vi "PicoScope4000aExampleRapidBlockBulkOverlapped.vi"() -> ()   [LabVIEW 2010]
doc: "This example demonstrates how to use the PicoScope Labview library to collect data using rapid block mode, retrieving the data values in bulk."
uses:
  shared/PicoBuffers.ctl
  PicoScope4000aLib/PicoScope4000aAnalogChannelSettings.ctl
  shared/Segment Range.ctl
  shared/Buffer and Transfer Settings.ctl
  shared/Acquisition Settings.ctl
  shared/nSegments.ctl
panel:
  in  "Resolution":u32(ring)=1 items=["8-bit", "12-bit", "14-bit"]
  out "Unit Info":T1
  in  "Trigger Settings":T2={"Trigger Enabled"=FALSE, "Trigger Source"=enum."Channel A", "Trigger Threshold (Volts/Probe units)"=0.0, "Trigger Direction"=2, "Trigger Delay (samples)"=0, "Auto Trigger Time (ms)"=1000} {"Trigger Direction" items=["Rising"=2, "Falling"=3]}
  out "overflow":i16[](array[numeric]) format="%08b"
  in  "Channel A Settings":T3={"Enabled"=TRUE, "Coupling"=1, "Range"=6, "Analogue Offset"=0.0, "Bandwidth Limit"=0} {"Bandwidth Limit" items=["Full", "20kHz", "100kHz", "1MHz"]; "Range" items=["10 mV", "20 mV", "50 mV", "100 mV", "200 mV", "500 mV", "1 V", "2 V", "5 V", "10 V", "20 V", "50 V ", "100 V"]; "Coupling" items=["AC", "DC"]}
  out "USB 3.0 device on non-USB 3.0 Port":bool
  out "USB Powered":bool=TRUE
  in  "Stop Display":bool
  out "Capture Complete":bool
  in  "Run":bool
  in  "Display Buffer Index":i32
  in  "Segment Range":T4={"fromSegmentIndex"=0, "toSegmentIndex"=9} {"toSegmentIndex" format="%.4p"; "fromSegmentIndex" format="%.4p"}
  in  "nSegments":T5=10 format="%.4p"
  out "error out":errorcluster
  in  "Data file":path=path "PicoScope4000aExampleRapidBlock ChA Data"
  in  "Buffer and Transfer Settings":T6={"startIndex"=0, "Samples"=5000000, "Down Sample Ratio"=1, "Down-Sample Mode"=0} {"Down-Sample Mode" items=["RAW none"=2147483648, "None"=0, "Aggregate"=1, "Decimate"=2, "Average"=4]; "Down Sample Ratio" step=1; "Samples" format="%_6p"}
  in  "Acquisition Settings":T7={"preTriggerSamples"=0, "postTriggerSamples"=5000000, "timebase"=5} {"postTriggerSamples" format="%_6p"; "preTriggerSamples" format="%_6p"}
  out "Properties Panel":T8={"Sample Frequency"=41666668.0, "Sample Rate"=2.4000000209412065e-08, "Max Samples Available"=26843008, "Number of Samples"=0, "Total Capture Time (sec) "=0.0, "Max Total Capture Time Available (sec)"=0.6442322134971619} {"Max Total Capture Time Available (sec)" format="%.3p"; "Sample Frequency" format="%.6p"; "Sample Rate" format="%.3p"; "Max Samples Available" format="%_6p"; "Total Capture Time (sec)" format="%.3p"}
  in  "stop":bool
  out "Analog Channels":cluster{i32, dbl, "Data":dbl[]}[](graph)
  in  "Serial Number":string
  in  "Use Serial Number":bool
  in  "error in (no error)":errorcluster
  # "Number of\nSegments to Capture"
  # "Bit 0 = ChA"
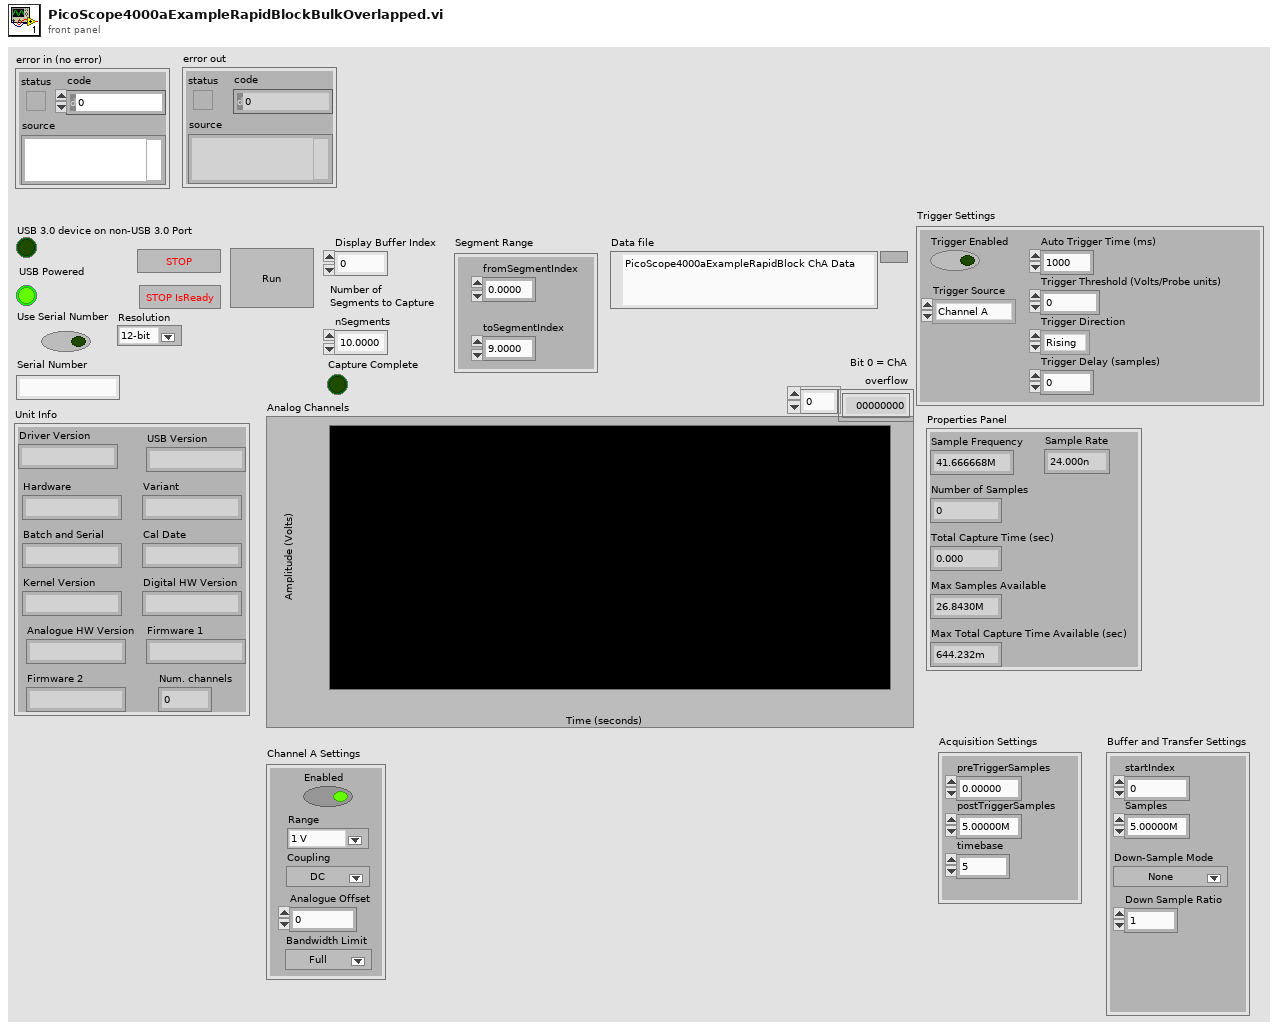
[diagram p1: front panel]
types:
  T1 = cluster{"Driver Version":string, "USB Version":string, "Hardware":string, "Variant":string, "Batch and Serial":string, "Cal Date":string, "Kernel Version":string, "Digital HW Version":string, "Analogue HW Version":string, "Firmware 1":string, "Firmware 2":string, "Num. channels":i16}
  T2 = cluster{"Trigger Enabled":bool, "Trigger Source":enum16{"Channel A", "Channel B", "Channel C", "Channel D", "Channel E", "Channel F", "Channel G", "Channel H"}, "Trigger Threshold (Volts/Probe units)":dbl, "Trigger Direction":u16, "Trigger Delay (samples)":u32, "Auto Trigger Time (ms)":i16}
  T3 = typedef "PicoScope4000aAnalogChannelSettings.ctl" = cluster{"Enabled":bool, "Coupling":i16, "Range":u16, "Analogue Offset":sgl, "Bandwidth Limit":u32}
  T4 = typedef "Segment Range.ctl" = cluster{"fromSegmentIndex":u64, "toSegmentIndex":u64}
  T5 = typedef "nSegments.ctl" = u64
  T6 = typedef "Buffer and Transfer Settings.ctl" = cluster{"startIndex":u64, "Samples":u64, "Down Sample Ratio":u64, "Down-Sample Mode":u32}
  T7 = typedef "Acquisition Settings.ctl" = cluster{"preTriggerSamples":u64, "postTriggerSamples":u64, "timebase":u32}
  T8 = cluster{"Sample Frequency":dbl, "Sample Rate":dbl, "Max Samples Available":u64, "Number of Samples":u64, "Total Capture Time (sec) ":dbl, "Max Total Capture Time Available (sec)":dbl}
  T9 = enum16{"open", "open or create", "create or replace", "create", "open (read-only)"}
  T10 = typedef "PicoBuffers.ctl" = cluster{"Max Buffer Pointers":u64[][][], "Min Buffer Pointers":u64[][][], "StreamingDataInfo":cluster{"Channel":u32, "Down-Sample Mode":u32, "PICO_DATA_TYPE":enum32{"PICO_INT8_T", "PICO_INT16_T", "PICO_INT32_T", "PICO_UINT32_T", "PICO_INT64_T", ""}, "Samples":i32, "bufferIndex":u64, "startIndex":i32, "overflow":i16}[][]}
  T11 = cluster{"Channel A Buffer":i16[], "Channel B Buffer":i16[], "Channel C Buffer":i16[], "Channel D Buffer":i16[], "Channel E Buffer":i16[], "Channel F Buffer":i16[], "Channel G Buffer":i16[], "Channel H Buffer":i16[], "Port 0 Buffer":i16[], "Port 1 Buffer":i16[]}[]
  T12 = cluster{"Channel A Buffer":i16[], "Channel B Buffer":i16[], "Channel C Buffer":i16[], "Channel D Buffer":i16[], "Channel E Buffer":i16[], "Channel F Buffer":i16[], "Channel G Buffer":i16[], "Channel H Buffer":i16[], "Port 0 Buffer":i16[], "Port 1 Buffer":i16[]}
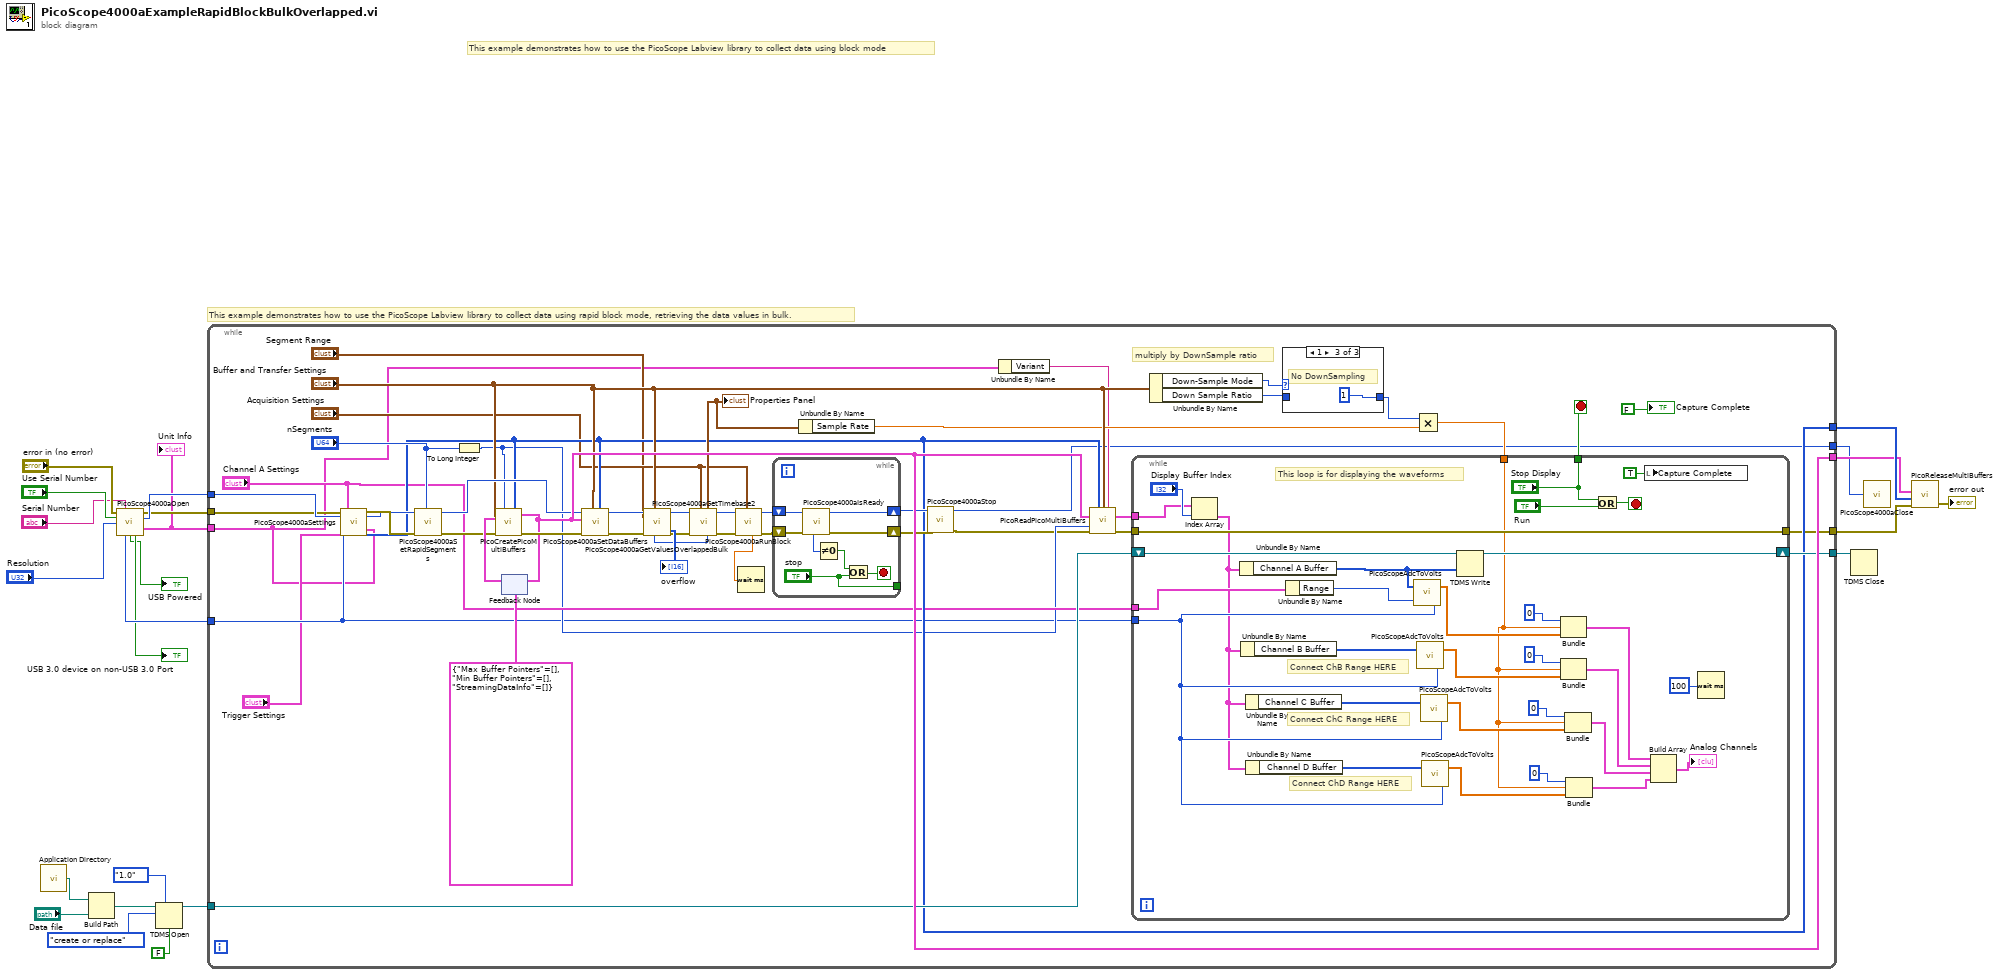
[diagram p0: block diagram]
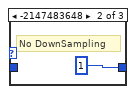
[diagram p3: hidden frame]
diagram:
  # "This example demonstrates how to use the PicoScope Labview library to collect data using rapid block mode, retrieving the data values in bulk."
  # "This example demonstrates how to use the PicoScope Labview library to collect data using block mode"
  n1 = call <vilib>:"Application Directory.vi"() -> ("Application Directory"=w14:path)
  n2 = Build Path(base path=w14, name or relative path="Data file") -> (appended path=w15:path)
  n3 = call "PicoScope4000aOpen.vi"("error in (no error)"="error in (no error)", "Serial Number"="Serial Number", "Use Serial Number"="Use Serial Number", "Resolution"="Resolution") -> ("error out"=w8:errorcluster, "handle"=w23:i16, "Unit Info"=w6:T1, "Max ADC value"=w9:i16, "USB powered"=→"USB Powered":bool, "USB 3.0 on non-USB 3.0 port"=→"USB 3.0 device on non-USB 3.0 Port":bool)  [unwired: 6 in]
  "Unit Info" <- w6
  n4 = TDMS Open(6:FALSE ("disable buffering? (T)"), 7:enum16{"1.0", "2.0"}."1.0" ("file format version (2.0)"), 10:T9."create or replace" ("operation (0:open)"), 11:w15) -> (3:w12:refnum<k34>)  [unwired: 2 in, 1 out]
  n5 = while {
    tunnel: w23 -> [w45]
    tunnel: w9 -> [w37]
    tunnel: [w26] -> w20
    tunnel: [w43] -> w22
    tunnel: [w69] -> w21
    tunnel: [w68] -> w13
    tunnel: w12 -> [w67]
    tunnel: w6 -> [w32]
    tunnel: w8 -> [w44]
    tunnel: [w42] -> w7
    stop <- w52 stop-if-true
    # "multiply by DownSample ratio"
    n6 = call "PicoScope4000aSettings.vi"("error in"=w44, "handle in"=w45, "Max ADC value"=w37, "Trigger Settings"="Trigger Settings", "Channel A Settings"="Channel A Settings", "Unit Info"=w32) -> ("error out"=w47:errorcluster, "handle out"=w46:i16, "Enabled array"=w43:i16[])  [unwired: 11 in]
    n7 = call "PicoScope4000aSetRapidSegments.vi"("nSegments"="nSegments", "error in (no error)"=w47, "handle in"=w46) -> ("error out"=w66:errorcluster, "handle out"=w65:i16)  [unwired: 6 in, 1 out]
    n8 = To Long Integer(number="nSegments") -> (32bit integer=w40:i32)
    n9 = feedback #1(T10 {"Max Buffer Pointers"=[], "Min Buffer Pointers"=[], "StreamingDataInfo"=[]} ("Data Pointers")) -> (w71:T10)
    n10 = call "PicoCreatePicoMultiBuffers.vi"("Number of Buffers"=w40, "Buffer and Transfer Settings"="Buffer and Transfer Settings", "enabled array"=w43, "Data Pointers In"=w71, "error in (no error)"=w66) -> ("Data Pointers"=w69:T10, "error out"=w70:errorcluster)  [unwired: 9 in]
    n11 = feedback-in #1(w69) -> ()
    n12 = call "PicoScope4000aSetDataBuffers.vi"("enabled array"=w43, "Buffer and Transfer Settings"="Buffer and Transfer Settings", "error in (no error)"=w70, "Data Pointers In"=w69, "handle in"=w65) -> ("error out"=w64:errorcluster, "handle out"=w63:i16)  [unwired: 5 in]
    n13 = call "PicoScope4000aGetValuesOverlappedBulk.vi"("Segment Range"="Segment Range", "Buffer and Transfer Settings"="Buffer and Transfer Settings", "error in (no error)"=w64, "handle in"=w63) -> ("error out"=w30:errorcluster, "handle out"=w31:i16, "overflow"=→"overflow":i16[], "noOfSamples"=w25:u64)  [unwired: 4 in]
    n14 = call "PicoScope4000aGetTimebase2.vi"("Number of Samples"=w25, "Acquisition Settings"="Acquisition Settings", "error in (no error)"=w30, "handle in"=w31) -> ("error out"=w28:errorcluster, "handle out"=w29:i16, "Properties Panel"=w58:T8)  [unwired: 5 in]
    "Properties Panel" <- w58
    n15 = call "PicoScope4000aRunBlock.vi"("Acquisition Settings"="Acquisition Settings", "error in (no error)"=w28, "handle in"=w29) -> ("error out"=w55:errorcluster, "handle out"=w54:i16, "timeIndisposedMs"=w24:dbl)  [unwired: 5 in, 1 out]
    n16 = Wait (ms)(milliseconds to wait=w24) -> ()  [unwired: 1 out]
    n17 = while {
      shift-right: [w111] -> w49
      shift-left: w55 -> [w112]
      shift-right: [w110] -> w48
      shift-left: w54 -> [w109]
      tunnel: ["stop"] -> _
      stop <- w106 stop-if-true
      n18 = call "PicoScope4000aIsReady.vi"("error in (no error)"=w112, "handle in"=w109) -> ("error out"=w111:errorcluster, "handle out"=w110:i16, "ready"=w108:i16)  [unwired: 7 in]
      n19 = Not Equal To 0?(x=w108) -> (x != 0?=w107:bool)
      n20 = Or(x=w107, y="stop") -> (x .or. y?=w106:bool)
    }
    n21 = Unbundle By Name(w58) -> ("Sample Rate"=w35:dbl)
    n22 = call "PicoScope4000aStop.vi"("error in (no error)"=w49, "handle in"=w48) -> ("error out"=w27:errorcluster, "handle out"=w26:i16)  [unwired: 8 in]
    n23 = Unbundle By Name(w32) -> ("Variant"=w34:string)
    n24 = call "PicoReadPicoMultiBuffers.vi"("enabled array"=w43, "Buffer and Transfer Settings"="Buffer and Transfer Settings", "Variant"=w34, "Data Pointers"=w69, "No of Buffers"=w40, "error in (no error)"=w27) -> ("MultiBuffers (Max or non-aggregated)"=w61:T11, "error out"=w53:errorcluster)  [unwired: 7 in, 1 out]
    n25 = Unbundle By Name("Buffer and Transfer Settings") -> ("Down-Sample Mode"=w59:u32, "Down Sample Ratio"=w60:u64)
    n26 = case shown="1" w59 {
      tunnel: [w113 u64 1 ("Down Sample Ratio") u64 1 ("Down Sample Ratio")] -> w56
      tunnel: w60 -> [w113 _ _]
      frame Default {
      }
      frame -2147483648 {
        # "No DownSampling"
      }
      frame 1 {
        # "No DownSampling"
      }
    }
    n27 = Multiply(x=w56, y=w35) -> (x*y=w57:dbl)
    n28 = while {
      tunnel: w37 -> [w74]
      tunnel: "Channel A Settings" -> [w104]
      tunnel: w61 -> [w84]
      tunnel: w57 -> [w76]
      shift-right: [w103] -> w68
      shift-left: w67 -> [w102]
      tunnel: [w90] -> w42
      tunnel: w53 -> [w90]
      tunnel: ["Stop Display"] -> w52
      stop <- w87 stop-if-true
      # "This loop is for displaying the waveforms"
      # "Connect ChB Range HERE"
      # "Connect ChD Range HERE"
      # "Connect ChC Range HERE"
      n29 = Index Array(array=w84, index="Display Buffer Index") -> (element=w73:T12)
      n30 = Unbundle By Name(w73) -> ("Channel A Buffer"=w92:i16[])
      n31 = Unbundle By Name(w73) -> ("Channel B Buffer"=w98:i16[])
      n32 = Unbundle By Name(w73) -> ("Channel C Buffer"=w82:i16[])
      n33 = Unbundle By Name(w73) -> ("Channel D Buffer"=w78:i16[])
      n34 = Unbundle By Name(w104) -> ("Range"=w100:u16)
      n35 = call "PicoScopeAdcToVolts.vi"("Max_adc"=w74, "Range Index"=w100, "Data"=w92) -> ("Data"=w93:dbl[])
      n36 = call "PicoScopeAdcToVolts.vi"("Max_adc"=w74, "Data"=w98) -> ("Data"=w97:dbl[])  [unwired: 1 in]
      n37 = call "PicoScopeAdcToVolts.vi"("Max_adc"=w74, "Data"=w82) -> ("Data"=w81:dbl[])  [unwired: 1 in]
      n38 = call "PicoScopeAdcToVolts.vi"("Max_adc"=w74, "Data"=w78) -> ("Data"=w77:dbl[])  [unwired: 1 in]
      n39 = TDMS Write(0:w102, 9:w92) -> (4:w103:refnum<k34>)  [unwired: 4 in, 3 out]
      n40 = Bundle(0, w76, "Data"=w93) -> (w96:cluster{i32, dbl, "Data":dbl[]})  [unwired: 1 in]
      n41 = Bundle(0, w76, "Data"=w97) -> (w95:cluster{i32, dbl, "Data":dbl[]})  [unwired: 1 in]
      n42 = Bundle(0, w76, "Data"=w81) -> (w80:cluster{i32, dbl, "Data":dbl[]})  [unwired: 1 in]
      n43 = Bundle(0, w76, "Data"=w77) -> (w75:cluster{i32, dbl, "Data":dbl[]})  [unwired: 1 in]
      n44 = Or(x="Stop Display", y="Run") -> (x .or. y?=w87:bool)
      n45 = local write "Capture Complete"(TRUE ("Capture Complete")) -> ()
      n46 = Build Array(w96, w95, w80, w75) -> (→"Analog Channels":cluster{i32, dbl, "Data":dbl[]}[])
      n47 = Wait (ms)(milliseconds to wait=u32 100) -> ()  [unwired: 1 out]
    }
    "Capture Complete" <- FALSE ("Capture Complete")
  }
  n48 = TDMS Close(11:w13) -> ()  [unwired: 1 in, 2 out]
  n49 = call "PicoScope4000aClose.vi"("handle"=w20) -> ()
  n50 = call "PicoReleaseMultiBuffers.vi"("error in (no error)"=w7, "Enabled array"=w22, "Data Pointers"=w21) -> ("error out"=→"error out":errorcluster)  [unwired: 8 in]
